vi "KYFG Buffer Get Frame Index.vi"(8 "error in (no error)":errorcluster, 11 "buffHandle":u32) -> (0 "error out":errorcluster, 2 "frame index":i32, 3 "buffHandle out":u32)   [LabVIEW 2023, in "KYFGLib_lv.lvlib"]
doc: "KYFG_API int KYFG_BufferGetFrameIndex(BUFFHANDLE buffHandle);"
uses:
  KYFGLib_lv.lvlib
  KYFGLib.dll
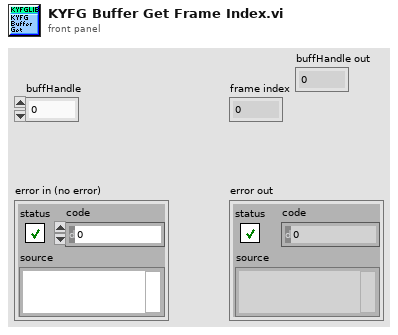
[diagram p1: front panel]
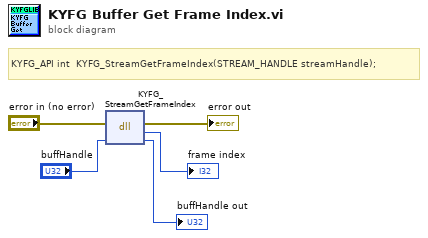
[diagram p0: block diagram]
diagram:
  # "KYFG_API int\t\tKYFG_StreamGetFrameIndex(STREAM_HANDLE streamHandle);"
  n1 = dll-call lib="KYFGLib.dll" fn="KYFG_StreamGetFrameIndex"(error in="error in (no error)", "streamHandle"="buffHandle") -> (error out=→"error out":errorcluster, "return type"=→"frame index":i32, "streamHandle"=→"buffHandle out":u32)  [unwired: 2 in, 1 out]
